vi "Check Last Write.vi"(8 "error in (no error)":errorcluster, 11 "Event Reporter Module in":refnum<class "Event Reporter Module.lvclass">) -> (0 "error out":errorcluster, 3 "Event Reporter Module out":refnum<class "Event Reporter Module.lvclass">)   [LabVIEW 2020, in "Volatus.lvlib" / "Event Reporter Module.lvclass"]
uses:
  Event Reporter Module.lvclass
  C:/dev/lv20CE/relink/lv-volatus/Volatus/Module/Module.lvclass
  Event Reporter Module.lvclass/Event Reporter Module.ctl
  Module/Module.lvclass/Module.ctl
  MessageQ/MessageQ.lvclass/MessageQ.ctl
  Module/Self Q.vi
  MessageQ/Send.vi
  Module/Module.lvclass
  C:/dev/lv20CE/relink/lv-volatus/Volatus/Event Reporter Module/Event Reporter Module.lvclass
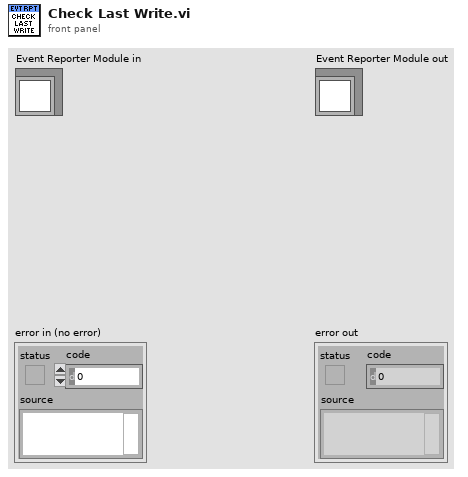
[diagram p1: front panel]
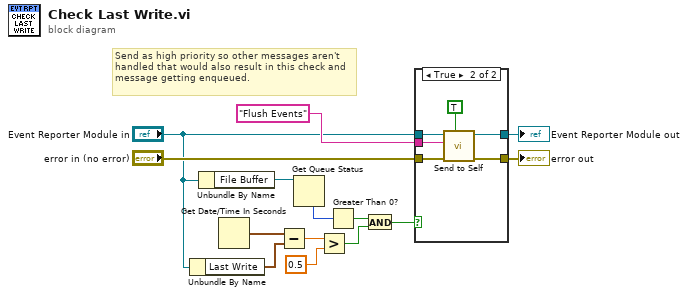
[diagram p0: block diagram]
diagram:
  # "Send as high priority so other messages aren't handled that would also result in this check and message getting enqueued."
  n1 = Unbundle By Name("Event Reporter Module in") -> ("Last Write"=w12:timestamp)
  n2 = Unbundle By Name("Event Reporter Module in") -> ("File Buffer"=w5:refnum<queue>)
  n3 = Get Date/Time In Seconds() -> (seconds since 1Jan1904=w13:timestamp)
  n4 = Subtract(x=w13, y=w12) -> (x-y=w11:dbl)
  n5 = Get Queue Status(queue=w5) -> (# elements in queue=w4:i32)  [unwired: 2 in, 7 out]
  n6 = Greater?(x=w11, y=0.5) -> (0:w2:bool)
  n7 = Greater Than 0?(x=w4) -> (x > 0?=w3:bool)
  n8 = And(x=w3, y=w2) -> (x .and. y?=w1:bool)
  n9 = case shown="True" w1 {
    tunnel: "error in (no error)" -> [w16 w22]
    tunnel: [w16 w18] -> w9
    tunnel: "Event Reporter Module in" -> [w15 w21]
    tunnel: [w15 w19] -> w8
    tunnel: "Flush Events" ("Message ID") -> [_ w20]
    frame False {
    }
    frame True {
      n10 = call "Send to Self.vi"("High Priority (F)"=TRUE, "error in (no error)"=w22, "Message ID"=w20, "Module in"=w21) -> ("error out"=w18:errorcluster, "Module out"=w19:refnum<class "Event Reporter Module.lvclass">)  [unwired: 6 in]
    }
  }
  "error out" <- w9
  "Event Reporter Module out" <- w8
